vi "GetAllInfo.vi"(0 "reference in":refnum<class "ClassRelationshipEdge.lvclass">, 5 "error in (no error)":errorcluster) -> (14 "reference out":refnum<class "ClassRelationshipEdge.lvclass">, 16 "AllInfo":T2, 17 "PathInfo":T1, 19 "error out":errorcluster)   [LabVIEW 2020, in "ClassRelationshipEdge.lvclass"]
uses:
  <resource>/Framework/Providers/Open_GDS/UML/ClassRelationshipEdge_class/ClassRelationshipEdge.lvclass
  C:/Program Files (x86)/National Instruments/LabVIEW 2020/resource/Framework/Providers/Open_GDS/UML/SegmentedLineEdge_class/SegmentedLineEdge.lvclass
  C:/Program Files (x86)/National Instruments/LabVIEW 2020/resource/Framework/Providers/Open_GDS/UML/AbstractEdge_class/AbstractEdge.lvclass
  <resource>/Framework/Providers/Open_GDS/UML/ClassRelationshipEdge_class/GetAllInfoType.ctl
  <resource>/Framework/Providers/Open_GDS/UML/AbstractNode_class/AbstractNode.lvclass
  <resource>/Framework/Providers/Open_GDS/UML/LineStyle_class/LineStyleType.ctl
  <resource>/Framework/Providers/Open_GDS/UML/ArrowHead_class/ArrowHeadType.ctl
  <resource>/Framework/Providers/Open_GDS/UML/ClassRelationshipEdge_class/PathInfoType.ctl
  <resource>/Framework/Providers/Open_GDS/UML/BentStyle_class/BentStyle.lvclass
  <resource>/Framework/Providers/Open_GDS/UML/LineStyle_class/LineStyle.lvclass
  <resource>/Framework/Providers/Open_GDS/UML/ArrowHead_class/ArrowHead.lvclass
  <resource>/Framework/Providers/Open_GDS/UML/SegmentedLineEdge_class/SegmentedLineEdge.lvclass
  <resource>/Framework/Providers/Open_GDS/UML/AbstractEdge_class/AbstractEdge.lvclass
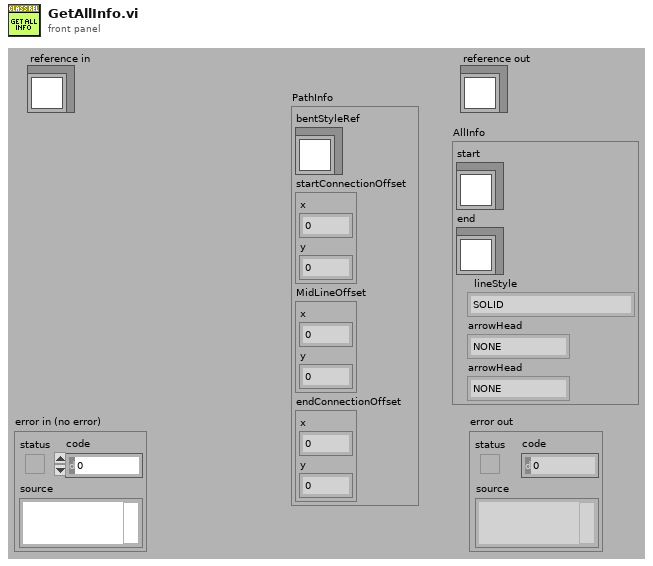
[diagram p1: front panel]
types:
  T1 = typedef "ClassRelationshipEdge.lvclass/PathInfoType.ctl" = cluster{"bentStyleRef":refnum<class "BentStyle.lvclass">, "startConnectionOffset":cluster{"x":i32, "y":i32}, "MidLineOffset":cluster{"x":i32, "y":i32}, "endConnectionOffset":cluster{"x":i32, "y":i32}}
  T2 = typedef "ClassRelationshipEdge.lvclass/GetAllInfoType.ctl" = cluster{"start":refnum<class "AbstractNode.lvclass">, "end":refnum<class "AbstractNode.lvclass">, "lineStyle":T3, "arrowHead":T4, "arrowHead":T4}
  T3 = typedef "LineStyle.lvclass/LineStyleType.ctl" = enum16{"SOLID", "DOTTED"}
  T4 = typedef "ArrowHead.lvclass/ArrowHeadType.ctl" = enum16{"NONE", "TRIANGLE", "BLACK_TRIANGLE", "V", "HALF_V", "DIAMOND", "BLACK_DIAMOND"}
  T5 = typedef "ClassRelationshipEdge.lvclass/ObjectAttributes.ctl" = cluster{"bentStyleRef":refnum<class "BentStyle.lvclass">, "startConnectionOffset":cluster{"x":i32, "y":i32}, "endConnectionOffset":cluster{"x":i32, "y":i32}, "MidLineOffset":cluster{"x":i32, "y":i32}, "DepClass":T6}
  T6 = typedef "ReversedEngineering_ViDependencyDetailsType.ctl" = cluster{"ThisVIs/Ctls":path[], "Dependent_VIs/Ctls":path[]}
  T7 = typedef "SegmentedLineEdge.lvclass/ObjectAttributes.ctl" = cluster{"lineStyle":refnum<class "LineStyle.lvclass">, "startArrowHead":refnum<class "ArrowHead.lvclass">, "endArrowHead":refnum<class "ArrowHead.lvclass">, "startLabel":string, "midLabel":string, "endLabel":string, "MidLabelOffset":T8, "SplitWire":bool}
  T8 = typedef "Point Point2D.ctl" = cluster{"x":dbl, "y":dbl}
  T9 = typedef "AbstractEdge.lvclass/ObjectAttributes.ctl" = cluster{"start":refnum<class "AbstractNode.lvclass">, "end":refnum<class "AbstractNode.lvclass">}
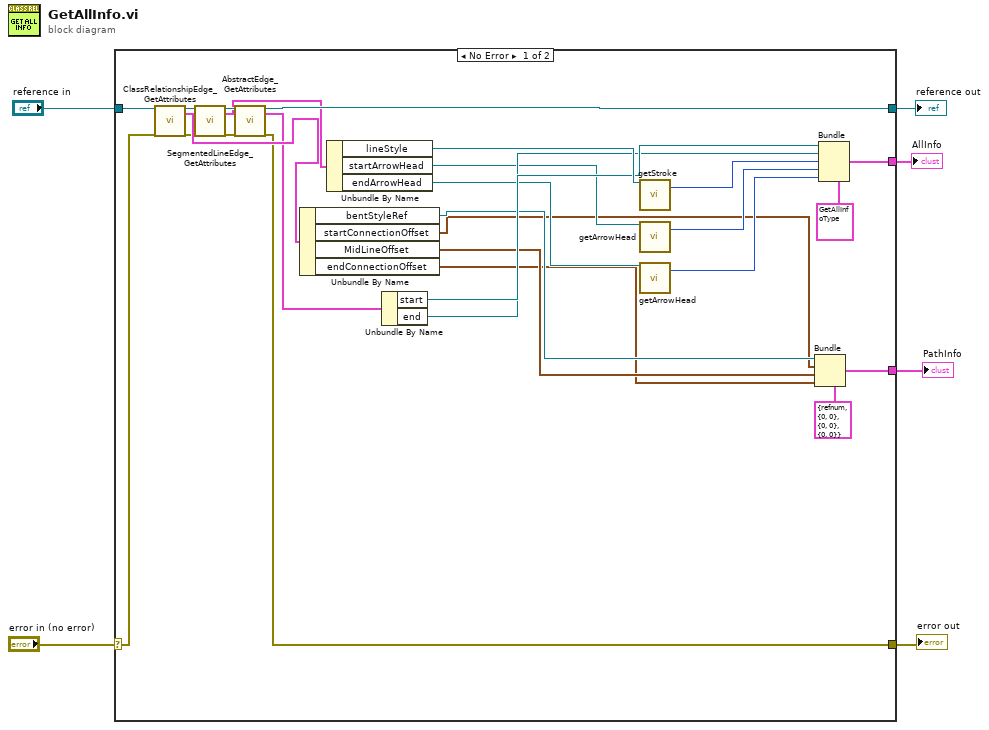
[diagram p0: block diagram]
diagram:
  n1 = case shown="No Error" "error in (no error)" {
    selector: "error in (no error)" -> [w33 w35]
    tunnel: [w10 w35] -> w5
    tunnel: [w9 w34] -> w3
    tunnel: "reference in" -> [w32 w34]
    tunnel: [w22 _] -> w2
    tunnel: [w19 _] -> w1
    frame No Error {
      n2 = call <resource>:"ClassRelationshipEdge_GetAttributes.vi"("reference in"=w32, "error in (no error)"=w33) -> ("reference out"=w14:refnum<class "ClassRelationshipEdge.lvclass">, "Data"=w15:T5, "error out"=w13:errorcluster)  [unwired: 14 in, 1 out]
      n3 = call <resource>:"SegmentedLineEdge_GetAttributes.vi"("reference in"=w14, "error in (no error)"=w13) -> ("reference out"=w12:refnum<class "ClassRelationshipEdge.lvclass">, "Data"=w7:T7, "error out"=w11:errorcluster)  [unwired: 14 in, 1 out]
      n4 = call <resource>:"AbstractEdge_GetAttributes.vi"("reference in"=w12, "error in (no error)"=w11) -> ("reference out"=w9:refnum<class "ClassRelationshipEdge.lvclass">, "Data"=w8:T9, "error out"=w10:errorcluster)  [unwired: 14 in, 1 out]
      n5 = Unbundle By Name(w15) -> ("bentStyleRef"=w21:refnum<class "BentStyle.lvclass">, "startConnectionOffset"=w20:cluster{"x":i32, "y":i32}, "MidLineOffset"=w18:cluster{"x":i32, "y":i32}, "endConnectionOffset"=w17:cluster{"x":i32, "y":i32})
      n6 = Unbundle By Name(w7) -> ("lineStyle"=w31:refnum<class "LineStyle.lvclass">, "startArrowHead"=w27:refnum<class "ArrowHead.lvclass">, "endArrowHead"=w25:refnum<class "ArrowHead.lvclass">)
      n7 = Unbundle By Name(w8) -> ("start"=w30:refnum<class "AbstractNode.lvclass">, "end"=w29:refnum<class "AbstractNode.lvclass">)
      n8 = call-dynamic "getStroke.vi"("reference"=w31) -> ("lineStyle"=w28:T3)  [unwired: 16 in, 2 out]
      n9 = call <resource>:"getArrowHead.vi"("reference"=w27) -> ("arrowHead"=w26:T4)  [unwired: 16 in, 2 out]
      n10 = call <resource>:"getArrowHead.vi"("reference"=w25) -> ("arrowHead"=w24:T4)  [unwired: 16 in, 2 out]
      n11 = Bundle(cluster=T1 {"bentStyleRef"=refnum, "startConnectionOffset"={"x"=0, "y"=0}, "MidLineOffset"={"x"=0, "y"=0}, "endConnectionOffset"={"x"=0, "y"=0}} ("PathInfo"), "bentStyleRef"=w21, "startConnectionOffset"=w20, "MidLineOffset"=w18, "endConnectionOffset"=w17) -> (w19:T1)
      n12 = Bundle(cluster=T2 {"start"=refnum, "end"=refnum, "lineStyle"=enum."SOLID", "arrowHead"=enum."NONE", "arrowHead"=enum."NONE"} ("output cluster"), "start"=w30, "end"=w29, "lineStyle"=w28, "arrowHead"=w26, "arrowHead"=w24) -> (w22:T2)
    }
    frame Error {
    }
  }
  "error out" <- w5
  "reference out" <- w3
  "AllInfo" <- w2
  "PathInfo" <- w1
